vi "Fetch Python Version.vi"(11 "Test Case In":refnum<class "Support VIs.lvclass">) -> (0 "error out":errorcluster, 3 "Test Case Out":refnum<class "Support VIs.lvclass">)   [LabVIEW 2026, in "Support VIs.lvclass"]
doc: "Check automatic fetching of python version. The corresponding python environment must exist in the relative location of the project."
uses:
  Support VIs.lvclass
  C:/Program Files/National Instruments/LabVIEW 2026/vi.lib/Astemes/LUnit/Test Case.lvclass
  <vilib>/Astemes/LUnit/Test Case.lvclass/Test Case.ctl
  <vilib>/Astemes/LUnit/Core/LUnit Test Case/Private/Append Fail Result.vi
  <vilib>/Astemes/LUnit/Core/LUnit Test Case/Private/Append Pass Result.vi
  <vilib>/Astemes/LUnit/Core/LUnit Test Case/Private/Run In UI.vi
  <vilib>/Utility/error.llb/Clear Errors.vi
  <vilib>/regexp/Match Regular Expression.xnode
  Support VIs.lvclass/Support VIs.ctl
  <vilib>/Astemes/LUnit/Test Case.lvclass
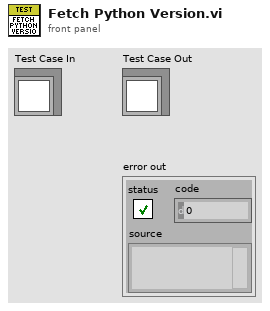
[diagram p1: front panel]
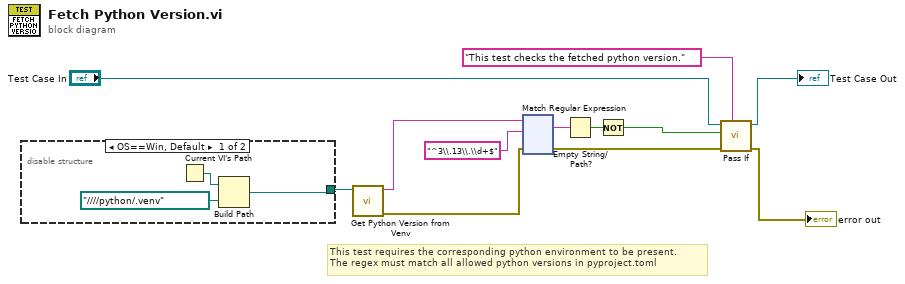
[diagram p0: block diagram]
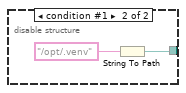
[diagram p2: hidden frame]
diagram:
  # "This test requires the corresponding python environment to be present.\nThe regex must match all allowed python versions in pyproject.toml"
  n1 = disable-structure shown="OS==Win, Default" {
    disable-tunnel: [w13 w17] -> w12
    frame condition #0 (active) {
      n2 = Current VI's Path() -> (path=w15:path)
      n3 = Build Path(base path=w15, name or relative path=path "../../../../python/.venv") -> (appended path=w13:path)
    }
    frame condition #1 {
      n4 = String To Path(string="/opt/.venv") -> (path=w17:path)
    }
  }
  n5 = call "Get Python Version from Venv.vi"("venv"=w12) -> ("error out"=w9:errorcluster, "Python Version"=w10:string)  [unwired: 9 in]
  n6 = xnode "Match Regular Expression"("input string"=w10, "regular expression"="^3\\.13\\.\\d+$", "error in"=w9) -> ("whole match"=w3:string, "error out"=w6:errorcluster)  [unwired: 3 in, 3 out]
  n7 = Empty String/Path?(string/path=w3) -> (empty?=w2:bool)
  n8 = Not(x=w2) -> (.not. x?=w1:bool)
  n9 = call <vilib>:"Pass If.vi"("Description"="This test checks the fetched python version.", "error in (no error)"=w6, "Pass?"=w1, "LUnit Test Case In"="Test Case In") -> ("error out"=→"error out":errorcluster, "LUnit Test Case Out"=→"Test Case Out":refnum<class "Support VIs.lvclass">)  [unwired: 6 in]
